vi "LvaiDialogProbe.vi"   [LabVIEW 2026]
doc: "Shows a modal One Button Dialog at startup and blocks until the dialog is dismissed. Used to probe how a modal dialog blocks an MCP run call."
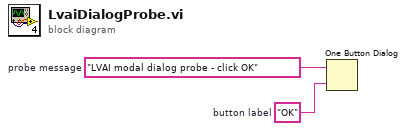
[diagram p0: block diagram]
diagram:
  w1 = "OK"  # button label
  w2 = "LVAI modal dialog probe - click OK"  # probe message
  n1 = One Button Dialog(message=w2, button name ("OK")=w1) -> ()  [unwired: 1 out]
